vi "KYFG Load Pattern Data.vi"(8 "error in (no error)":errorcluster, 9 "patternType":i32, 10 "streamHandle":u32) -> (0 "error out":errorcluster, 2 "streamHandle out":u32)   [LabVIEW 2023]
doc: "KYFG_API FGSTATUS KYFG_SetCameraValue(CAMHANDLE camHandle, const char *paramName, void *paramValue);"
uses:
  KYFGLib_lv.lvlib
  KYFGLib.dll
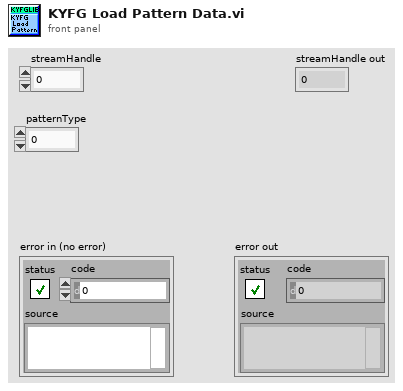
[diagram p1: front panel]
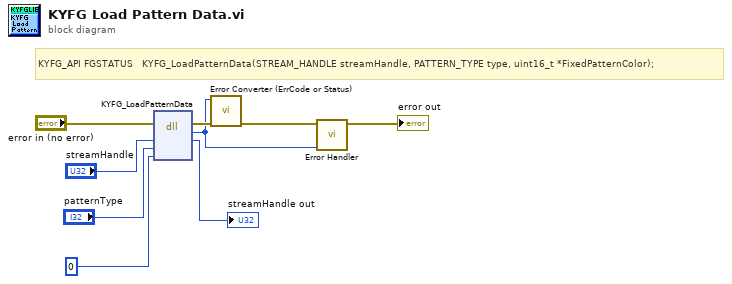
[diagram p0: block diagram]
diagram:
  # "KYFG_API FGSTATUS   KYFG_LoadPatternData(STREAM_HANDLE streamHandle, PATTERN_TYPE type, uint16_t *FixedPatternColor);"
  n1 = dll-call lib="KYFGLib.dll" fn="KYFG_LoadPatternData"(error in="error in (no error)", "streamHandle"="streamHandle", "patternType"="patternType", "fixedPatternValue"=u16 0 ("fixedPatternData")) -> (error out=w7:errorcluster, "return type"=w6:u32, "streamHandle"=→"streamHandle out":u32)  [unwired: 4 in, 1 out]
  n2 = call "Error Converter (ErrCode or Status).vi"("error in (no error)"=w7, "error code"=w6) -> ("error out"=w5:errorcluster)  [unwired: 9 in]
  n3 = call "Error Handler.vi"("Return Code"=w6, "Error In"=w5) -> ("Error Out"=→"error out":errorcluster)  [unwired: 9 in]
